vi "XIS Is Correction Ready.vi"(8 "error in (no error)":errorcluster, 10 "gainReady":i32, 11 "offsetReady":i32) -> (0 "error out":errorcluster, 1 "function return":i32, 2 "gainReady out":i32, 3 "offsetReady out":i32)   [LabVIEW 2022 SP3, in "VarexWrapper.lvlib"]
doc: "VAREX_API int XIS_IsCorrectionReady(int* offsetReady, int* gainReady);"
uses:
  VarexWrapper.lvlib
  VarexWrapper.dll
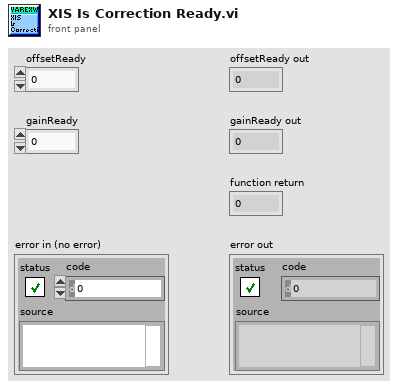
[diagram p1: front panel]
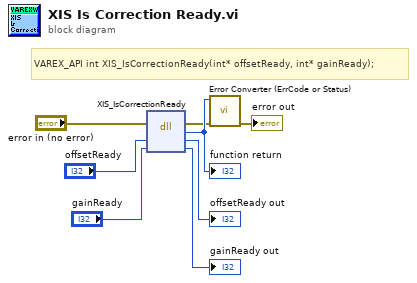
[diagram p0: block diagram]
diagram:
  # "VAREX_API int XIS_IsCorrectionReady(int* offsetReady, int* gainReady);"
  n1 = dll-call lib="E:/SourceCodes/image-harvest/ImageHandler/VarexWrapperLvLib/VarexWrapper.*" fn="XIS_IsCorrectionReady"(error in="error in (no error)", "offsetReady"="offsetReady", "gainReady"="gainReady") -> (error out=w2:errorcluster, w8:i32, "offsetReady"=→"offsetReady out":i32, "gainReady"=→"gainReady out":i32)  [unwired: 2 in, 1 out]
  "function return" <- w8
  n2 = call "Error Converter (ErrCode or Status).vi"("error in (no error)"=w2, "error code"=w8) -> ("error out"=→"error out":errorcluster)  [unwired: 9 in]
